vi "Read master instance.vi"(8 "error in (no error)":errorcluster, 11 "Modbus_Master in":refnum<class "Modbus_Master.lvclass">) -> (0 "error out":errorcluster, 2 "Modbus Master":refnum<class "Modbus Master.lvclass">, 3 "Modbus_Master out":refnum<class "Modbus_Master.lvclass">)   [LabVIEW 2021, in "Modbus_Master.lvclass"]
uses:
  Modbus_Master.lvclass
  <vilib>/NI/Modbus Library/API/Master/Modbus Master.lvclass
  Modbus_Master.lvclass/Modbus_Master.ctl
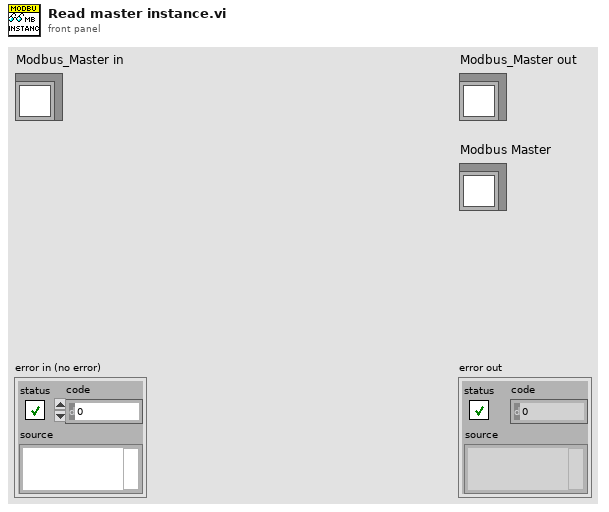
[diagram p1: front panel]
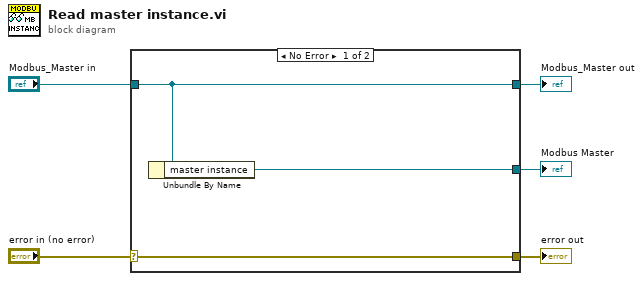
[diagram p0: block diagram]
diagram:
  n1 = case shown="No Error" "error in (no error)" {
    selector: "error in (no error)" -> [w8 w9]
    tunnel: [w8 w9] -> w4
    tunnel: [w7 w10] -> w2
    tunnel: "Modbus_Master in" -> [w7 w10]
    tunnel: [w6 _] -> w1
    frame No Error {
      n2 = Unbundle By Name(w7) -> ("master instance"=w6:refnum<class "Modbus Master.lvclass">)
    }
    frame Error {
    }
  }
  "error out" <- w4
  "Modbus_Master out" <- w2
  "Modbus Master" <- w1
